vi "meas_mult_2021.vi"() -> ()   [LabVIEW 2019]
uses:
  <instrlib>/Agilent 3446X Series/Public/Data/Read (Single Point).vi
  <instrlib>/Agilent 3446X Series/Agilent 3446X Series.lvlib
panel:
  in  "Measurement Function (10: Voltage DC)":i32(ring)=10 items=["Continuity", "Current AC", "Current DC", "Diode", "Frequency", "Resistance 4-wire", "Period", "Resistance 2-wire", "Temperature", "Voltage AC", "Voltage DC", "Voltage DC Ratio", "Capacitance"]
  out "Measurement":dbl
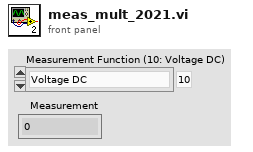
[diagram p1: front panel]
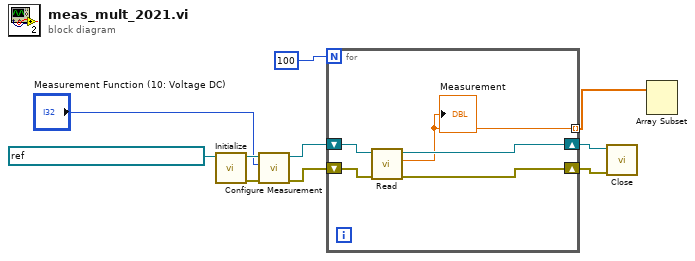
[diagram p0: block diagram]
diagram:
  n1 = call <instrlib>:"Initialize.vi"("VISA resource name"=refnum<visa-resource-name> "TCPIP0::192.168.2.4::inst0::INSTR") -> ("error out"=w10:errorcluster, "VISA resource name out"=w7:refnum<visa-resource-name>)  [unwired: 9 in]
  n2 = call <instrlib>:"Configure Measurement.vi"("error in (no error)"=w10, "Measurement Function (10: Voltage DC)"="Measurement Function (10: Voltage DC)", "VISA resource name"=w7) -> ("error out"=w4:errorcluster, "VISA resource name out"=w5:refnum<visa-resource-name>)  [unwired: 7 in]
  n3 = for {
    N: 100 -> [_]
    shift-right: [w14] -> w8
    shift-left: w5 -> [w13]
    shift-right: [w15] -> w9
    shift-left: w4 -> [w12]
    tunnel: [w11] -> w1 mode=indexing
    n4 = call-poly <instrlib>:"Read.vi"("error in (no error)"=w12, "VISA resource name"=w13) -> ("error out"=w15:errorcluster, "Measurement"=w11:dbl, "VISA resource name out"=w14:refnum<visa-resource-name>)  [unwired: 7 in]
    "Measurement" <- w11
  }
  n5 = call <instrlib>:"Close.vi"("error in (no error)"=w9, "VISA resource name"=w8) -> ()  [unwired: 9 in, 1 out]
  n6 = Array Subset "Array Subset"(array=w1) -> ()  [unwired: 2 in, 1 out]
